vi "CSM_Bookmarks_Refs.vi"(8 "error in (no error)":errorcluster, 11 "VIRef":refnum<vi>) -> (0 "error out":errorcluster, 2 "Array":cluster{refnum<vi>, "Text":string}[](array[cluster]), 3 "Reference Out":refnum<vi>)   [LabVIEW 2017]
uses:
  _csmHelper/Utility/_Support/Diagram.llb/csmHelper-Diagram.lvlib
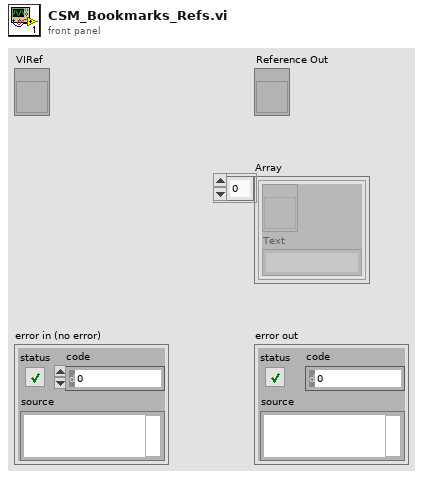
[diagram p1: front panel]
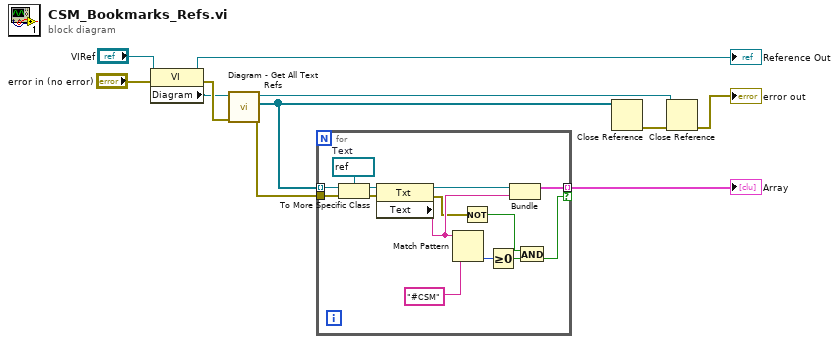
[diagram p0: block diagram]
diagram:
  n1 = property on="Property Node" class="VI"(reference="VIRef", error in="error in (no error)") -> (reference out=→"Reference Out":refnum<vi>, error out=w11:errorcluster, "Diagram"=w3:refnum<vi>)
  n2 = call "Diagram - Get All Text Refs.vi"("error in (no error)"=w11, "TopLevelDiagram in"=w3) -> ("error out"=w4:errorcluster, "TextRefs"=w1:refnum<vi>[], "TopLevelDiagram out"=w2:refnum<vi>)  [unwired: 7 in]
  n3 = for {
    tunnel: w1 -> [w25] mode=indexing
    tunnel: w4 -> [w24]
    tunnel: [w18] -> w5 mode=indexing if=w14
    w23 = refnum<vi> refnum  # Text
    n4 = To More Specific Class(target class=w23, reference=w25, error in=w24) -> (specific class reference=w22:refnum<vi>, error out=w20:errorcluster)
    n5 = property class="Txt"(reference=w22, error in=w20) -> (reference out=w21:refnum<vi>, error out=w13:errorcluster, "Text"=w17:string)
    n6 = Match Pattern(string=w17, regular expression="#CSM") -> (offset past match=w16:i32)  [unwired: 1 in, 3 out]
    n7 = Not(x=w13) -> (.not. x?=w12:bool)
    n8 = Greater Or Equal To 0?(x=w16) -> (x >= 0?=w15:bool)
    n9 = Bundle(w21, "Text"=w17) -> (w18:cluster{refnum<vi>, "Text":string})  [unwired: 1 in]
    n10 = And(x=w12, y=w15) -> (x .and. y?=w14:bool)
  }
  "Array" <- w5
  n11 = Close Reference(reference=w1) -> (error out=w10:errorcluster)  [unwired: 1 in]
  n12 = Close Reference(reference=w2, error in (no error)=w10) -> (error out=→"error out":errorcluster)
